vi "Populate Serial Channels.vi"(8 "error in (no error)":errorcluster, 10 "Strings []":string[](array[string]), 11 "SERIAL INPUT (SI) Ref in":refnum<vi>) -> (0 "error out":errorcluster, 3 "SERIAL INPUT (SI) Ref out":refnum<vi>)   [LabVIEW 2025, in "I2C Bus Monitor UI.lvlib"]
uses:
  I2C Bus Monitor UI.lvlib
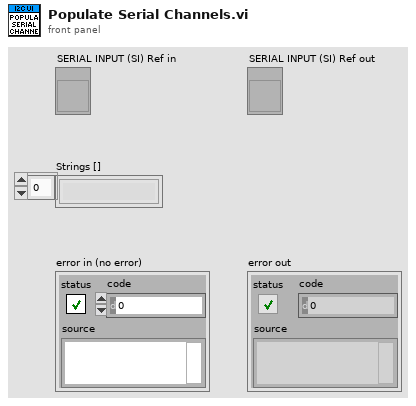
[diagram p1: front panel]
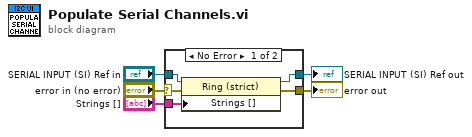
[diagram p0: block diagram]
diagram:
  n1 = case shown="No Error" "error in (no error)" {
    selector: "error in (no error)" -> [w9 w11]
    tunnel: "SERIAL INPUT (SI) Ref in" -> [w10 w12]
    tunnel: "Strings []" -> [w8 _]
    tunnel: [w7 w11] -> w2
    tunnel: [w6 w12] -> w1
    frame No Error {
      n2 = property on="Property Node" class="Ring (strict)"(reference=w10, error in=w9, "Strings []"=w8) -> (reference out=w6:refnum<vi>, error out=w7:errorcluster)
    }
    frame Error {
    }
  }
  "error out" <- w2
  "SERIAL INPUT (SI) Ref out" <- w1
